vi "1d.peak_wavelength.vi"() -> ()   [LabVIEW 2017]
uses:
  <vilib>/Instr/_visa.llb/VISA Configure Serial Port (Instr).vi
panel:
  out "Measured peak wavelengths":dbl[](array[numeric]) format="%.3g"
  out "Peak amplitudes":dbl[](array[numeric])
  out "Waveform Graph":dbl[](graph)
  out "XY Graph":T1(graph)
  in  "Stop":bool
  in  "Integration time (µs) 2":i32=100000
  out "read buffer 2":string
  out "VISA resource name out":refnum<visa-resource-name>
  out "read buffer":string
  in  "VISA resource name":refnum<visa-resource-name>="COM3" caption="Serial COM port"
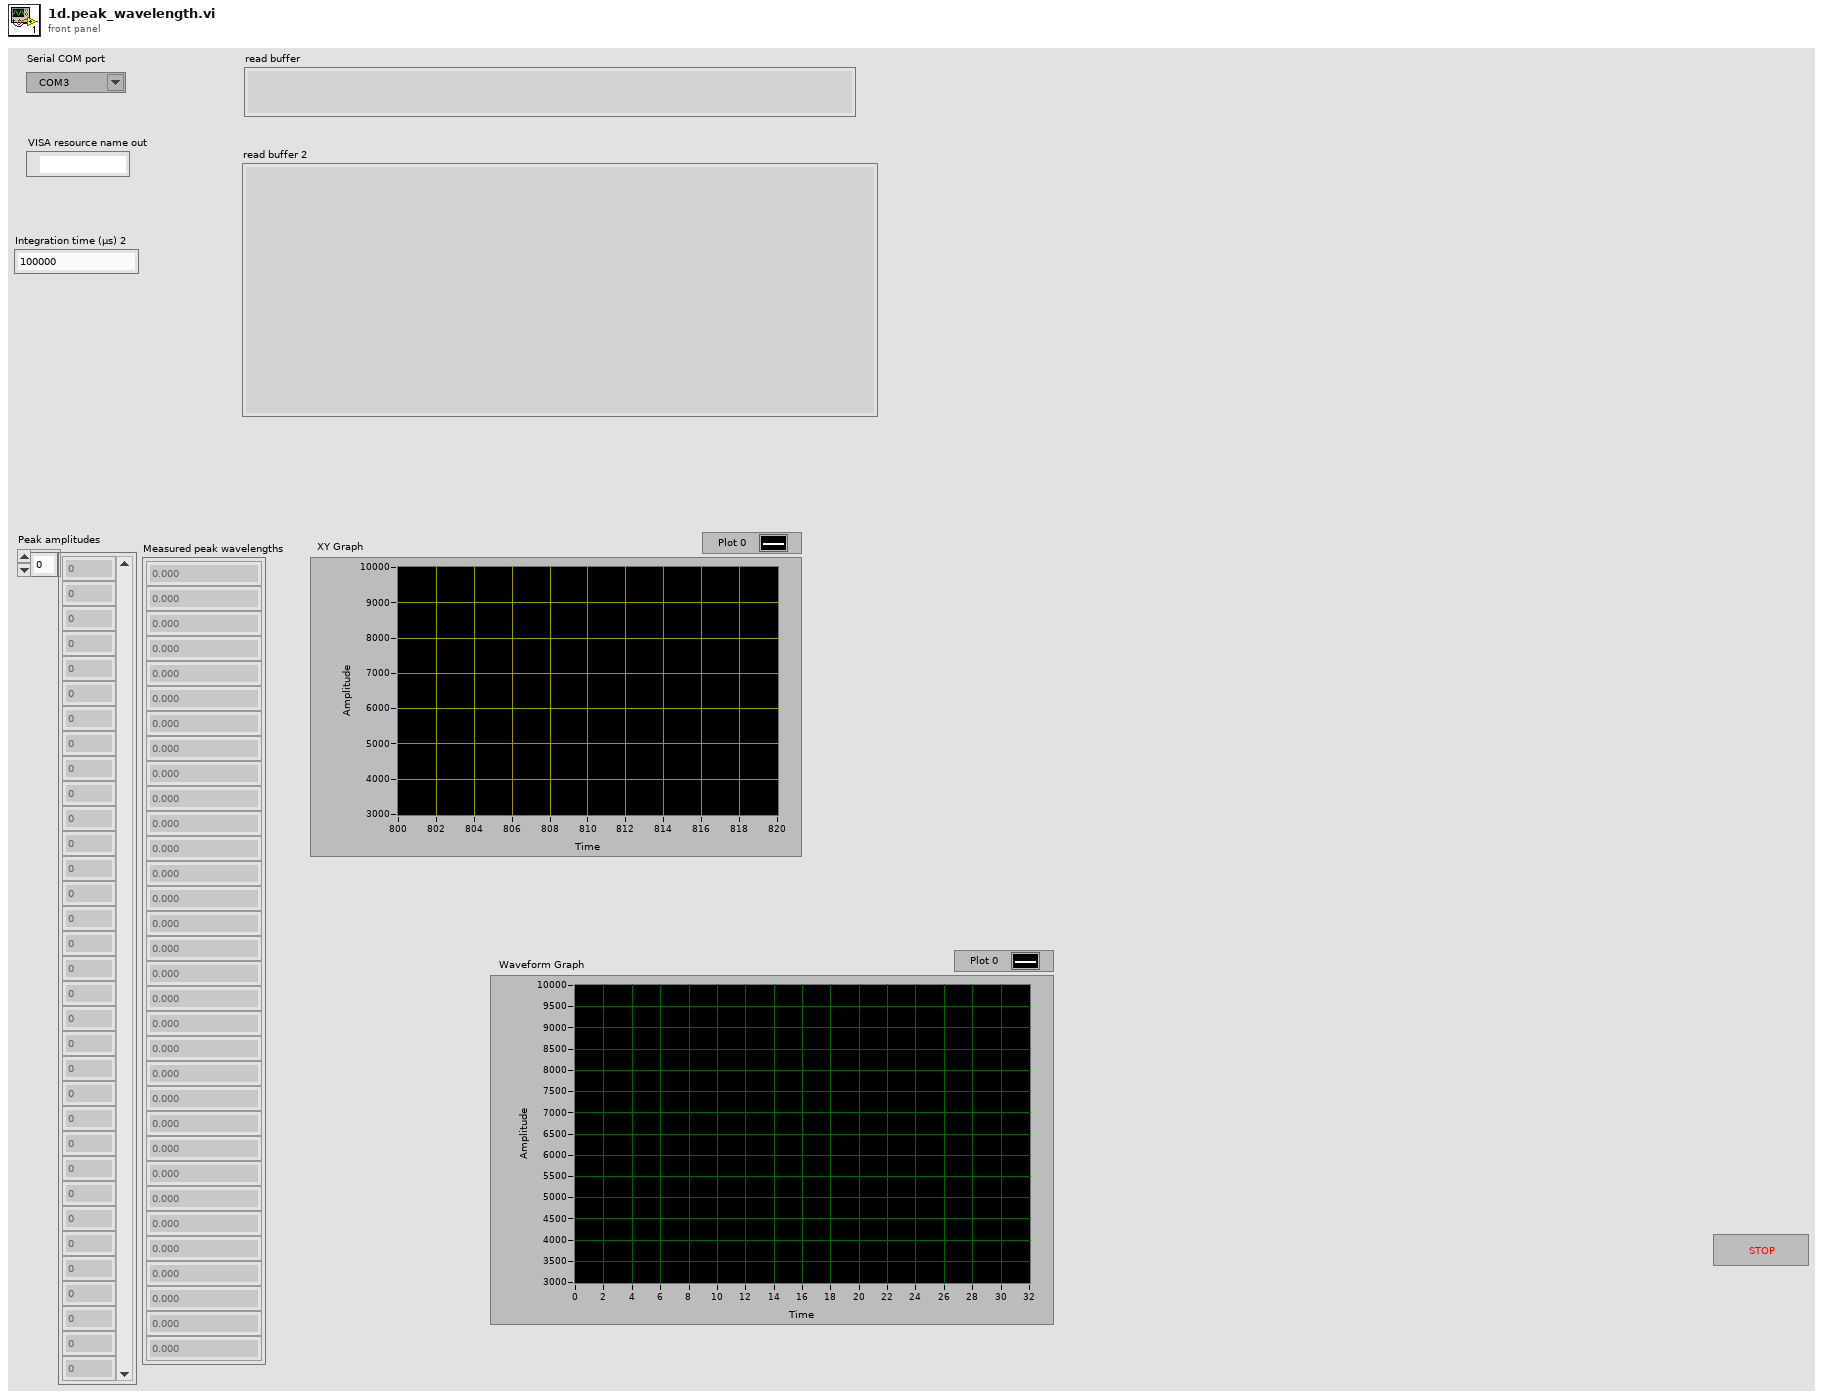
[diagram p1: front panel]
types:
  T1 = cluster{"Peak wavelengths":dbl[], "Peak amplitudes":dbl[]}
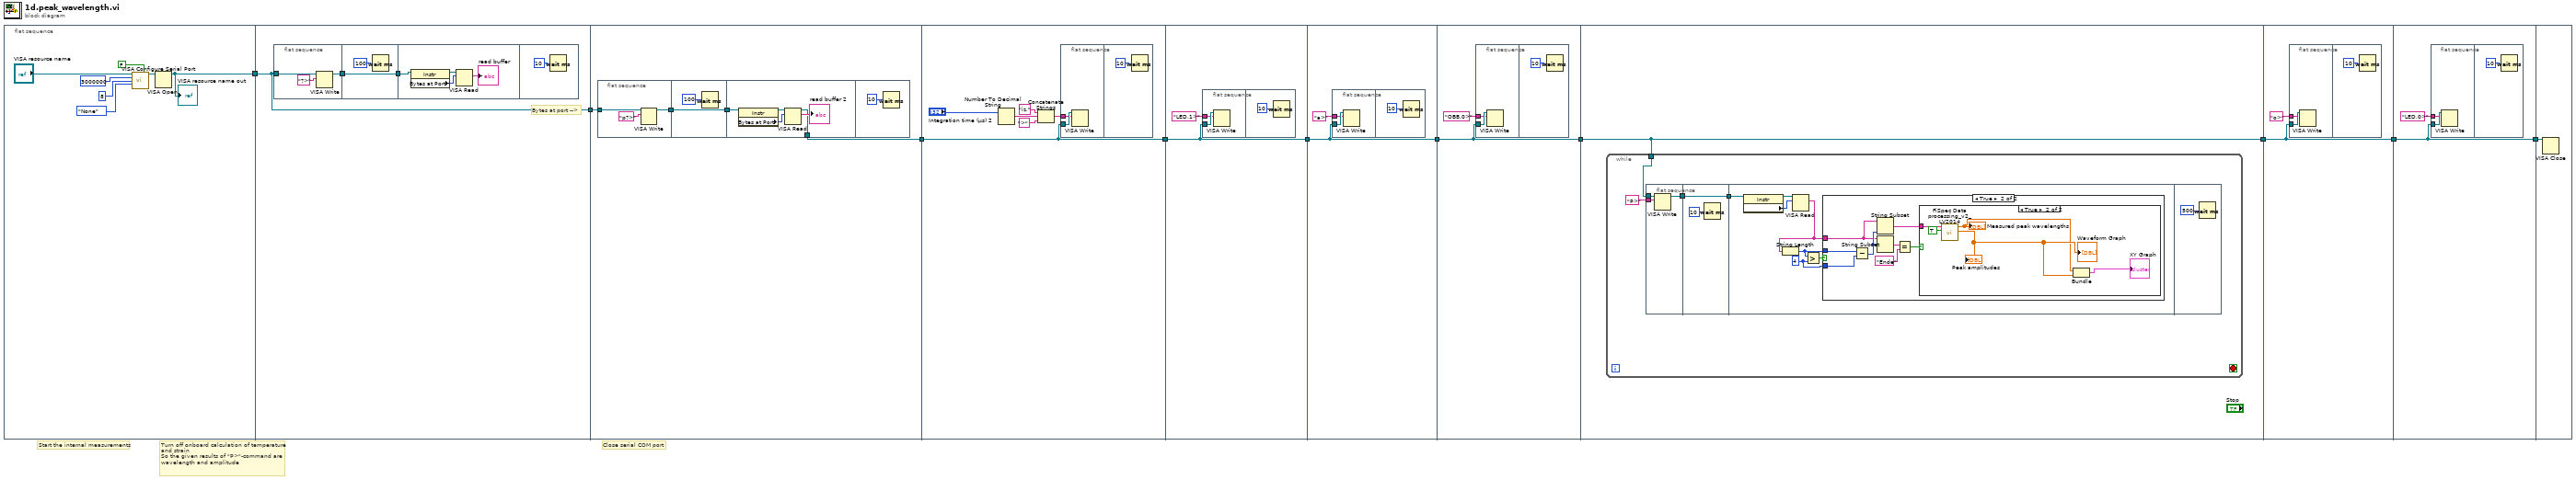
[diagram p0: block diagram]
diagram:
  # "Turn off onboard calculation of temperature and strain\nSo the given results of \"P>\"-command are wavelength and amplitude"
  # "Close serial COM port"
  # "Start the internal measurements"
  n1 = flat-sequence {
    tunnel: [w13] -> w10
    tunnel: w10 -> [w18]
    tunnel: [w18] -> w9
    tunnel: w9 -> [w32]
    tunnel: [w31] -> w8
    tunnel: w8 -> [w46]
    tunnel: [w46] -> w7
    tunnel: w7 -> [w55]
    tunnel: [w55] -> w6
    tunnel: w6 -> [w60]
    tunnel: [w60] -> w5
    tunnel: w5 -> [w65]
    tunnel: [w65] -> w4
    tunnel: w4 -> [w70]
    tunnel: [w70] -> w3
    tunnel: w3 -> [w101]
    tunnel: [w101] -> w2
    tunnel: w2 -> [w106]
    tunnel: [w106] -> w1
    tunnel: w1 -> [w111]
    frame #0 {
      n2 = call-poly "VISA Configure Serial Port"("VISA resource name"="VISA resource name", "Enable Termination\nChar (T)"=FALSE ("Enable Termination\nChar (T)"), "baud rate (9600)"=u32 3000000, "data bits (8)"=u16 8, "parity (0:none)"=enum16{"None", "Odd", "Even", "Mark", "Space"}."None") -> ("VISA resource name out"=w17:refnum<visa-resource-name>)  [unwired: 9 in, 1 out]
      n3 = VISA Open(VISA resource name=w17) -> (VISA resource name=w13:refnum<visa-resource-name>)  [unwired: 4 in, 1 out]
      "VISA resource name out" <- w13
    }
    frame #1 {
      # "Bytes at port -->"
      n4 = flat-sequence {
        tunnel: [w23] -> w20
        tunnel: w18 -> [w22]
        tunnel: [w24] -> w19
        tunnel: w20 -> [w24]
        tunnel: w19 -> [w29]
        frame #0 {
          n5 = VISA Write(VISA resource name=w22, write buffer="?>") -> (VISA resource name out=w23:refnum<visa-resource-name>)  [unwired: 1 in, 2 out]
        }
        frame #1 {
          n6 = Wait (ms)(milliseconds to wait=u32 100 ("Zu wartende ms")) -> ()  [unwired: 1 out]
        }
        frame #2 {
          n7 = property class="Instr"(reference=w29) -> (reference out=w28:refnum<visa-resource-name>, "Bytes at Port"=w27:u32)  [unwired: 1 in, 1 out]
          n8 = VISA Read(VISA resource name=w28, byte count=w27) -> (read buffer=→"read buffer":string)  [unwired: 1 in, 3 out]
        }
        frame #3 {
          n9 = Wait (ms)(milliseconds to wait=u32 10 ("Zu wartende ms")) -> ()  [unwired: 1 out]
        }
      }
    }
    frame #2 {
      n10 = flat-sequence {
        tunnel: [w37] -> w34
        tunnel: w32 -> [w35]
        tunnel: [w38] -> w33
        tunnel: w34 -> [w38]
        tunnel: w33 -> [w44]
        tunnel: [w40] -> w31
        frame #0 {
          n11 = VISA Write(VISA resource name=w35, write buffer="p?>") -> (VISA resource name out=w37:refnum<visa-resource-name>)  [unwired: 1 in, 2 out]
        }
        frame #1 {
          n12 = Wait (ms)(milliseconds to wait=u32 100 ("Zu wartende ms")) -> ()  [unwired: 1 out]
        }
        frame #2 {
          n13 = property class="Instr"(reference=w44) -> (reference out=w43:refnum<visa-resource-name>, "Bytes at Port"=w42:u32)  [unwired: 1 in, 1 out]
          n14 = VISA Read(VISA resource name=w43, byte count=w42) -> (VISA resource name out=w40:refnum<visa-resource-name>, read buffer=→"read buffer 2":string)  [unwired: 1 in, 2 out]
        }
        frame #3 {
          n15 = Wait (ms)(milliseconds to wait=u32 10 ("Zu wartende ms")) -> ()  [unwired: 1 out]
        }
      }
    }
    frame #3 {
      n16 = Number To Decimal String(number="Integration time (µs) 2") -> (decimal integer string=w51:string)  [unwired: 1 in]
      n17 = Concatenate Strings("iz," ("String"), w51, ">" ("String")) -> (w48:string)
      n18 = flat-sequence {
        tunnel: w46 -> [w53]
        tunnel: w48 -> [w52]
        frame #0 {
          n19 = VISA Write(VISA resource name=w53, write buffer=w52) -> ()  [unwired: 1 in, 3 out]
        }
        frame #1 {
          n20 = Wait (ms)(milliseconds to wait=u32 10 ("Zu wartende ms")) -> ()  [unwired: 1 out]
        }
      }
    }
    frame #4 {
      n21 = flat-sequence {
        tunnel: w55 -> [w58]
        tunnel: "LED,1>" ("String") -> [w57]
        frame #0 {
          n22 = VISA Write(VISA resource name=w58, write buffer=w57) -> ()  [unwired: 1 in, 3 out]
        }
        frame #1 {
          n23 = Wait (ms)(milliseconds to wait=u32 10 ("Zu wartende ms")) -> ()  [unwired: 1 out]
        }
      }
    }
    frame #5 {
      n24 = flat-sequence {
        tunnel: w60 -> [w63]
        tunnel: "a>" ("String") -> [w62]
        frame #0 {
          n25 = VISA Write(VISA resource name=w63, write buffer=w62) -> ()  [unwired: 1 in, 3 out]
        }
        frame #1 {
          n26 = Wait (ms)(milliseconds to wait=u32 10 ("Zu wartende ms")) -> ()  [unwired: 1 out]
        }
      }
    }
    frame #6 {
      n27 = flat-sequence {
        tunnel: w65 -> [w68]
        tunnel: "OBB,0>" ("String") -> [w67]
        frame #0 {
          n28 = VISA Write(VISA resource name=w68, write buffer=w67) -> ()  [unwired: 1 in, 3 out]
        }
        frame #1 {
          n29 = Wait (ms)(milliseconds to wait=u32 10 ("Zu wartende ms")) -> ()  [unwired: 1 out]
        }
      }
    }
    frame #7 {
      n30 = while {
        tunnel: w70 -> [w72]
        stop <- _ stop-if-true
        n31 = flat-sequence {
          tunnel: w72 -> [w77]
          tunnel: "P>" ("String") -> [w76]
          tunnel: [w75] -> w74
          tunnel: [w78] -> w73
          tunnel: w74 -> [w78]
          tunnel: w73 -> [w86]
          frame #0 {
            n32 = VISA Write(VISA resource name=w77, write buffer=w76) -> (VISA resource name out=w75:refnum<visa-resource-name>)  [unwired: 1 in, 2 out]
          }
          frame #1 {
            n33 = Wait (ms)(milliseconds to wait=u32 10 ("Zu wartende ms")) -> ()  [unwired: 1 out]
          }
          frame #2 {
            w81 = 4 ("y")
            n34 = property class="Instr"(reference=w86) -> (reference out=w85:refnum<visa-resource-name>, "Serial Settings:Number of Bytes at Serial Port"=w84:u32)  [unwired: 1 in, 1 out]
            n35 = VISA Read(VISA resource name=w85, byte count=w84) -> (read buffer=w80:string)  [unwired: 1 in, 3 out]
            n36 = String Length(string=w80) -> (length=w82:i32)
            n37 = Greater?(x=w82, y=w81) -> (0:w83:bool)
            n38 = case shown="True" w83 {
              tunnel: w80 -> [_ w91]
              tunnel: w82 -> [_ w89]
              tunnel: w81 -> [_ w88]
              frame False {
              }
              frame True {
                n39 = Subtract(x=w89, y=w88) -> (x-y=w92:i32)
                n40 = String Subset(string=w91, length (rest)=w92) -> (substring=w90:string)  [unwired: 1 in]
                n41 = String Subset(string=w91, offset (0)=w92) -> (substring=w94:string)  [unwired: 1 in]
                n42 = Equal?(x=w94, y="Ende") -> (x = y?=w87:bool)
                n43 = case shown="True" w87 {
                  tunnel: w90 -> [_ w99]
                  frame False {
                  }
                  frame True {
                    n44 = call "FiSpec Data processing_v2_LV2014.vi"("Onboard peak detection"=TRUE, "Data string (without \"Ende\")"=w99) -> ("Peak amplitudes"=w97:dbl[], "Peak wavelengths"=w96:dbl[])  [unwired: 4 in, 4 out]
                    "Measured peak wavelengths" <- w96
                    "Peak amplitudes" <- w97
                    "Waveform Graph" <- w97
                    n45 = Bundle("Peak wavelengths"=w96, "Peak amplitudes"=w97) -> (→"XY Graph":T1)  [unwired: 1 in]
                  }
                }
              }
            }
          }
          frame #3 {
            n46 = Wait (ms)(milliseconds to wait=u32 500 ("Zu wartende ms")) -> ()  [unwired: 1 out]
          }
        }
      }
    }
    frame #8 {
      n47 = flat-sequence {
        tunnel: w101 -> [w104]
        tunnel: "o>" ("String") -> [w103]
        frame #0 {
          n48 = VISA Write(VISA resource name=w104, write buffer=w103) -> ()  [unwired: 1 in, 3 out]
        }
        frame #1 {
          n49 = Wait (ms)(milliseconds to wait=u32 10 ("Zu wartende ms")) -> ()  [unwired: 1 out]
        }
      }
    }
    frame #9 {
      n50 = flat-sequence {
        tunnel: w106 -> [w109]
        tunnel: "LED,0>" ("String") -> [w108]
        frame #0 {
          n51 = VISA Write(VISA resource name=w109, write buffer=w108) -> ()  [unwired: 1 in, 3 out]
        }
        frame #1 {
          n52 = Wait (ms)(milliseconds to wait=u32 10 ("Zu wartende ms")) -> ()  [unwired: 1 out]
        }
      }
    }
    frame #10 {
      n53 = VISA Close(VISA resource name=w111) -> ()  [unwired: 1 in, 1 out]
    }
  }
